vi "PicoScope2000IsReady.vi"(8 "error in (no error)":errorcluster, 11 "handle in":i16) -> (0 "error out":errorcluster, 3 "handle out":i16, 6 "ready":i16)   [LabVIEW 2009]
doc: "Calls ps5000aIsReady"
uses:
  ps2000.dll
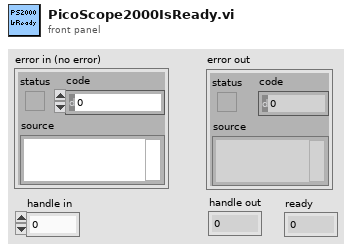
[diagram p1: front panel]
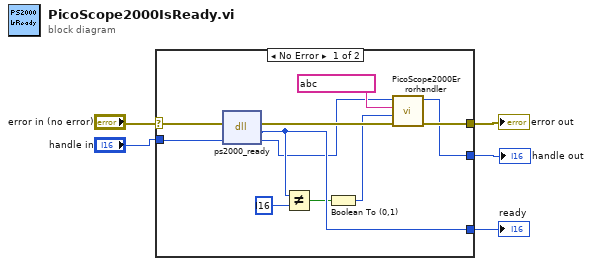
[diagram p0: block diagram]
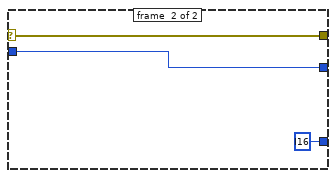
[diagram p2: hidden frame]
diagram:
  n1 = case shown="No Error" "error in (no error)" {
    selector: "error in (no error)" -> [w16 w18]
    tunnel: "handle in" -> [w15 w19]
    tunnel: [w8 w19] -> w5
    tunnel: [w12 w18] -> w4
    tunnel: [w14 i16 ? ("ready")] -> w3
    frame #0 {
      n2 = dll-call lib="PS2000.dll" fn="ps2000_ready"(error in=w16, "handle"=w15) -> (error out=w11:errorcluster, "return type"=w14:i16, "handle"=w9:i16)  [unwired: 2 in, 1 out]
      n3 = Not Equal?(x=w14, y=i16 ?) -> (x != y?=w7:bool)
      n4 = Boolean To (0,1)(Boolean=w7) -> (0, 1=w6:i16)
      n5 = call "PicoScope2000Errorhandler.vi"("Handle in"=w9, "API function"=string ?, "Return"=w6, "error in (no error)"=w11) -> ("Handle out"=w8:i16, "error out"=w12:errorcluster)  [unwired: 5 in]
    }
    frame #1 {
    }
  }
  "error out" <- w4
  "handle out" <- w5
  "ready" <- w3
